vi "Blit_Load.vi"(11 "error in":errorcluster) -> (4 "Sprites":cluster{"Pix":u8[][], "Mask":u8[][]}[](array[cluster]), 15 "error out":errorcluster)   [LabVIEW 2020, in "GH_Render.lvlib"]
doc: "Loads all sprites as raw pixels for Sprite_Blit: Resources\\Sprites\\sprites_blit.txt (Width;Height;Offset per sprite, order of sprites.txt) and sprites.bin (per sprite Height*Width*3 bytes RGB, then as many mask bytes, 255 = visible). Written by build\\make_blit.py."
uses:
  GH_Render.lvlib
  Level/GH_Level.lvlib
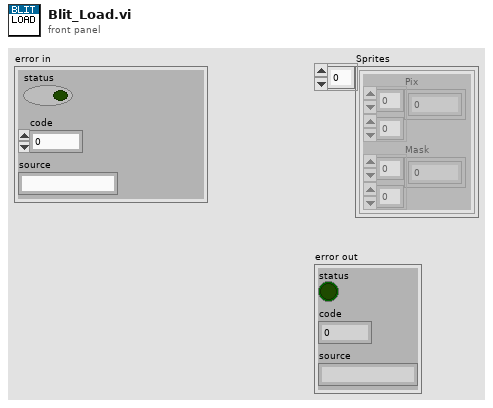
[diagram p1: front panel]
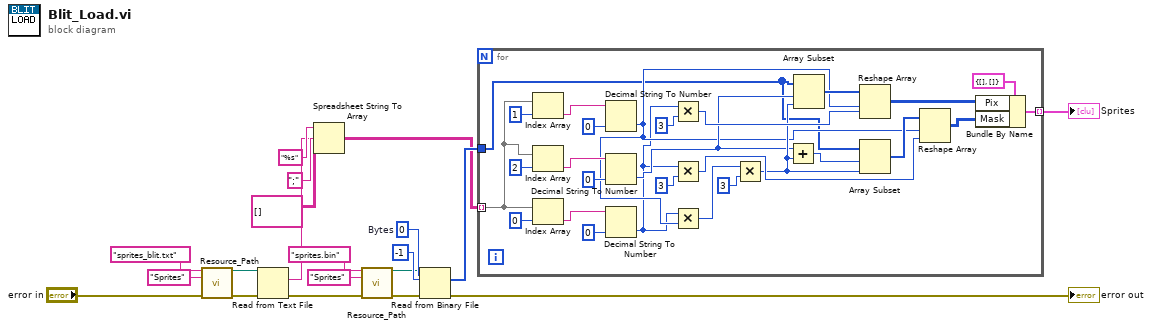
[diagram p0: block diagram]
diagram:
  w17 = u8 0  # Bytes
  n1 = call "Resource_Path.vi"("File name"="sprites_blit.txt", "Subfolder"="Sprites", "error in"="error in") -> ("Path"=w4:path, "error out"=w5:errorcluster)  [unwired: 11 in]
  n2 = Read from Text File(file (use dialog)=w4, error in=w5) -> (text=w6:string, error out=w7:errorcluster)  [unwired: 2 in, 2 out]
  n3 = Spreadsheet String To Array(delimiter (Tab)=";", format string="%s", spreadsheet string=w6, array type (2D Dbl)=string[][] []) -> (array=w11:string[][])
  n4 = call "Resource_Path.vi"("File name"="sprites.bin", "Subfolder"="Sprites", "error in"=w7) -> ("Path"=w14:path, "error out"=w15:errorcluster)  [unwired: 11 in]
  n5 = Read from Binary File(5:w17, 8:w15, 10:-1, 11:w14) -> (0:→"error out":errorcluster, 2:w18:u8[])  [unwired: 2 in, 2 out]
  n6 = for {
    tunnel: w11 -> [w21] mode=indexing
    tunnel: w18 -> [w22]
    tunnel: [w48] -> w20 mode=indexing
    n7 = Index Array(array=w21, index=1) -> (element=w28:string)
    n8 = Index Array(array=w21, index=2) -> (element=w32:string)
    n9 = Index Array(array=w21, index=0) -> (element=w24:string)
    n10 = Decimal String To Number(string=w28, default (0L)=0) -> (number=w30:i32)  [unwired: 1 in, 1 out]
    n11 = Decimal String To Number(string=w32, default (0L)=0) -> (number=w34:i32)  [unwired: 1 in, 1 out]
    n12 = Decimal String To Number(string=w24, default (0L)=0) -> (number=w26:i32)  [unwired: 1 in, 1 out]
    n13 = Multiply(x=w26, y=3) -> (x*y=w42:i32)
    n14 = Multiply(x=w26, y=3) -> (x*y=w45:i32)
    n15 = Multiply(x=w26, y=w30) -> (x*y=w35:i32)
    n16 = Multiply(x=w35, y=3) -> (x*y=w37:i32)
    n17 = Add(x=w34, y=w37) -> (x+y=w39:i32)
    n18 = Array Subset(array=w22, index=w34, length=w37) -> (w38:u8[])
    n19 = Reshape Array(w38, w30, w42) -> (w43:u8[][])
    n20 = Array Subset(array=w22, index=w39, length=w37) -> (w40:u8[])
    n21 = Reshape Array(w40, w30, w45) -> (w46:u8[][])
    n22 = Bundle By Name(cluster=cluster{"Pix":u8[][], "Mask":u8[][]} {"Pix"=[], "Mask"=[]}, "Pix"=w43, "Mask"=w46) -> (w48:cluster{"Pix":u8[][], "Mask":u8[][]})
  }
  "Sprites" <- w20
